vi "UI Merge Messsages into Map.vi"(8 "error in (no error)":errorcluster, 10 "pcap CAN DATA in":u8[](array[numeric]), 11 "CAN Return MAP in":T1 {"CAN frame"."payload" format="%x"; "CAN frame"."timestamp" format="%<%.7X\n%x>T"; "CAN frame"."type" items=["CAN Data"=0, "CAN Remote"=1, "CAN Bus Error"=2, "CAN 2.0 Data"=8, "CAN FD Data"=16, "CAN FD+BRS Data"=24, "J1939 Data"=192, "Delay"=224, "Log Trigger"=225, "Start Trigger"=226]; "CAN frame"."identifier" format="%x"}) -> (0 "error out":errorcluster, 3 "CAN Return MAP out":T1 {"CAN frame"."payload" format="%x"; "CAN frame"."timestamp" format="%<%.7X\n%x>T"; "CAN frame"."type" items=["CAN Data"=0, "CAN Remote"=1, "CAN Bus Error"=2, "CAN 2.0 Data"=8, "CAN FD Data"=16, "CAN FD+BRS Data"=24, "J1939 Data"=192, "Delay"=224, "Log Trigger"=225, "Start Trigger"=226]; "CAN frame"."identifier" format="%x"})   [LabVIEW 2021, in "XNET CAN RW.lvclass"]
doc: "Merge multiple CAN messages and only keep the last message for each ID. Intended for UI display."
uses:
  XNET CAN RW.lvclass
  typedef/CAN Return Map.ctl
  <vilib>/xnet/xnet.llb/XNET Frame CAN.ctl
  <vilib>/xnet/xnet.llb/XNET Frame Type CAN.ctl
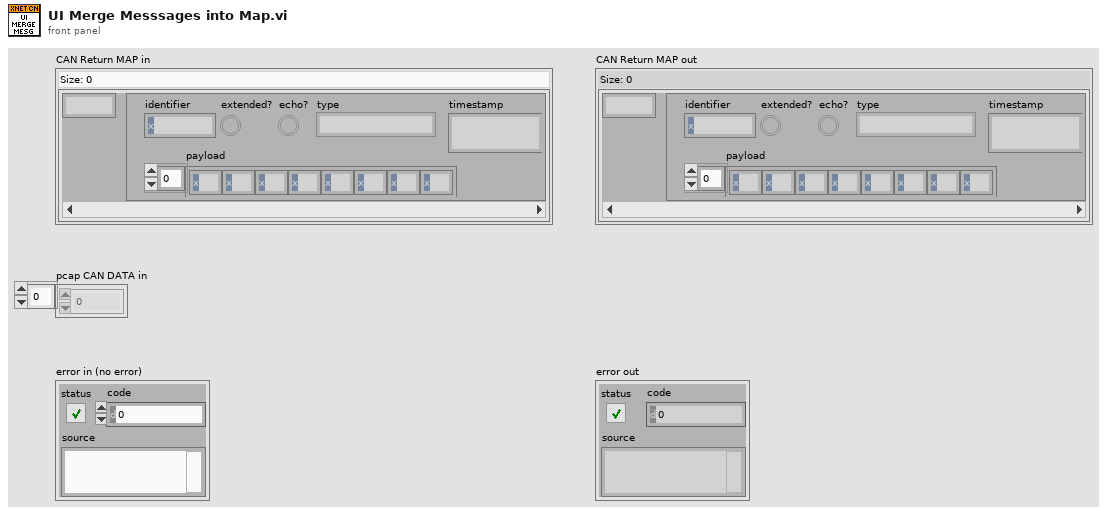
[diagram p1: front panel]
types:
  T1 = typedef "XNET CAN RW.lvclass/CAN Return Map.ctl" = map{u32, T2}
  T2 = typedef "XNET Frame CAN.ctl" = cluster{"timestamp":timestamp, "payload":u8[], "identifier":u32, "type":T3, "extended?":bool, "echo?":bool}
  T3 = typedef "XNET Frame Type CAN.ctl" = u8
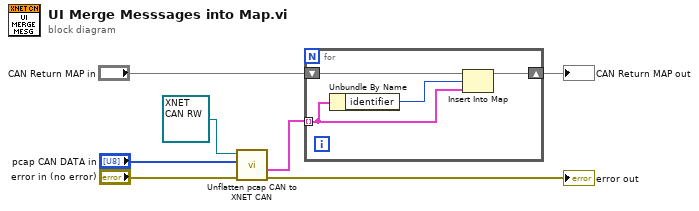
[diagram p0: block diagram]
diagram:
  n1 = call "Unflatten pcap CAN to XNET CAN.vi"("error in (no error)"="error in (no error)", "pcap CAN DATA in"="pcap CAN DATA in", "XNET_CAN_RW in"=refnum<class "XNET CAN RW.lvclass"> refnum) -> ("error out"=→"error out":errorcluster, "XNET CAN Data"=w4:T2[])  [unwired: 3 in, 4 out]
  n2 = for {
    tunnel: w4 -> [w9] mode=indexing
    shift-right: [w8] -> w1
    shift-left: "CAN Return MAP in" -> [w11]
    n3 = Unbundle By Name(w9) -> ("identifier"=w10:u32)
    n4 = Insert Into Map(map in=w11, key=w10, value=w9) -> (map out=w8:T1)  [unwired: 2 out]
  }
  "CAN Return MAP out" <- w1
